vi "set Peak Excursion.vi"(8 "error in (no error)":errorcluster caption="에러 입력(에러 없음)", 10 "Peak Excursion":dbl, 11 "FSV-40N 입력":refnum<class "FSV-40N.lvclass">) -> (0 "error out":errorcluster caption="에러 출력", 3 "FSV-40N 출력":refnum<class "FSV-40N.lvclass">)   [LabVIEW 2023, in "Spectrum Analyzer.lvlib" / "FSV-40N.lvclass"]
uses:
  FSV-40N.lvclass
  FSV-40N.lvclass/FSV-40N.ctl
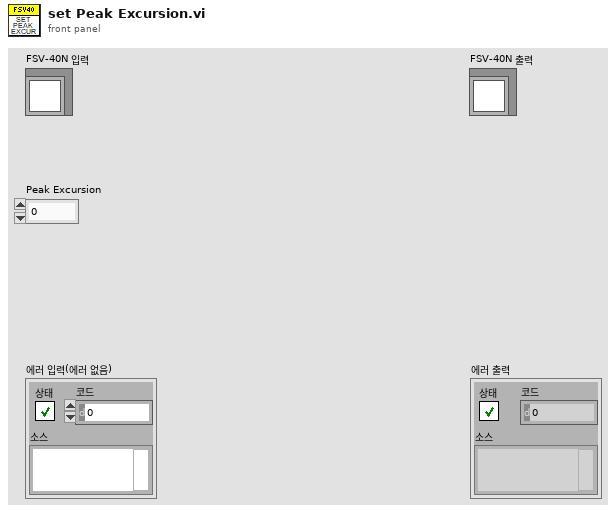
[diagram p1: front panel]
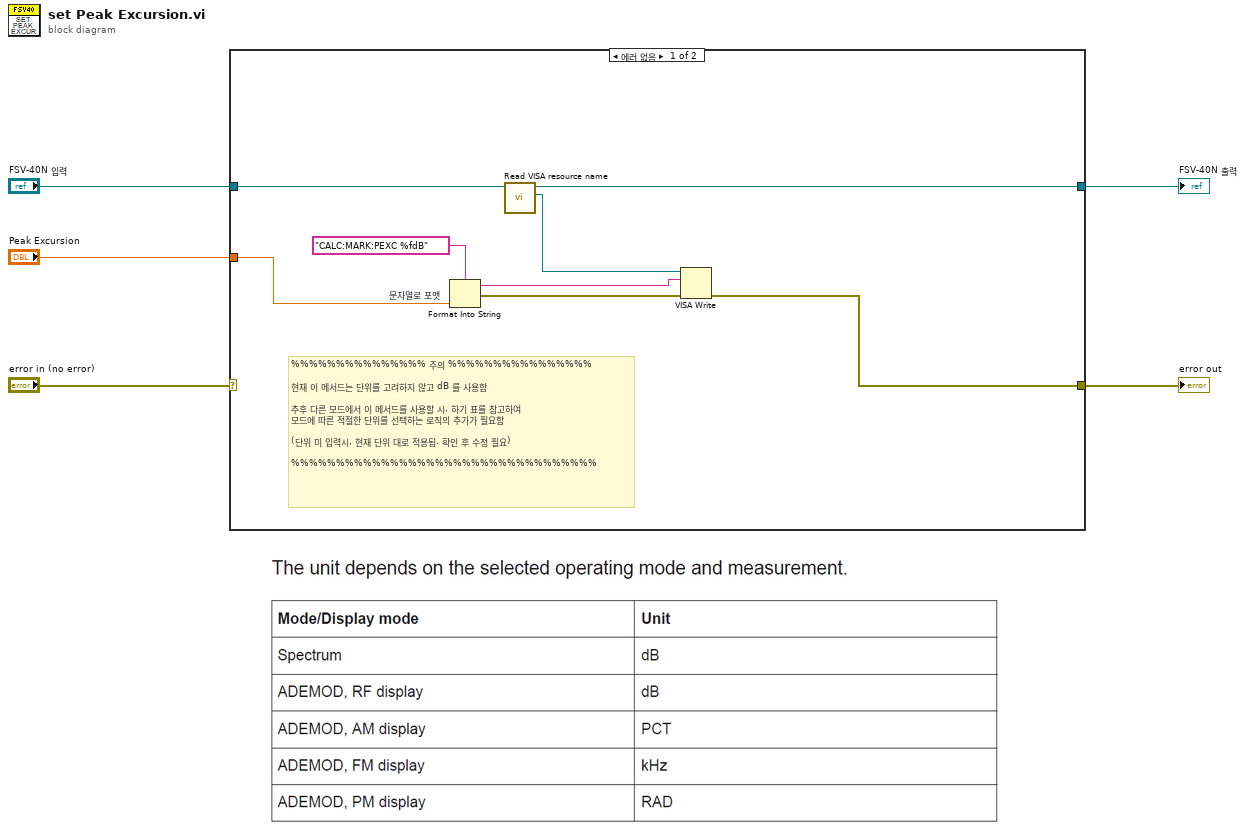
[diagram p0: block diagram]
diagram:
  n1 = case shown="에러 없음" "error in (no error)" {
    selector: "error in (no error)" -> [_ w14]
    tunnel: "FSV-40N 입력" -> [w12 w15]
    tunnel: [w8 w15] -> w3
    tunnel: [w7 w14] -> w2
    tunnel: "Peak Excursion" -> [w6 _]
    frame No Error {
      # "%%%%%%%%%%%%%%% 주의 %%%%%%%%%%%%%%%%\n\n현재 이 메서드는 단위를 고려하지 않고 dB 를 사용함\n\n추후 다른 모드에서 이 메서드를 사용할 시, 하기 표를 참고하여\n모드에 따른 적절한 단위를 선택하는 로직의 추가가 필요함\n\n(단위 미 입력시, 현재 단위 대로 적용됨. 확인 후 수정 필요)\n\n%%%%%%%%%%%%%%%%%%%%%%%%%%%%%%%%%%"
      n2 = Format Into String "문자열로 포맷"(format string="CALC:MARK:PEXC %fdB", w6) -> (resulting string=w9:string, error out=w11:errorcluster)  [unwired: 2 in]
      n3 = call "Read VISA resource name.vi"("FSV-40N in"=w12) -> ("VISA resource name"=w10:refnum<visa-resource-name>, "FSV-40N out"=w8:refnum<class "FSV-40N.lvclass">)  [unwired: 8 in, 1 out]
      n4 = VISA Write(VISA resource name=w10, write buffer=w9, error in (no error)=w11) -> (error out=w7:errorcluster)  [unwired: 2 out]
    }
    frame Error {
    }
  }
  "error out" <- w2
  "FSV-40N 출력" <- w3
